vi "SelectByUID.vi"(8 "error in (no error)":errorcluster, 10 "UID":i32, 11 "appended array":refnum<vi>[](array[refnum])) -> (0 "error out":errorcluster, 3 "GObject out":refnum<vi>)   [LabVIEW 2020]
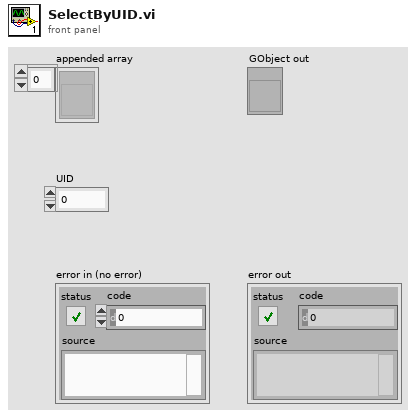
[diagram p1: front panel]
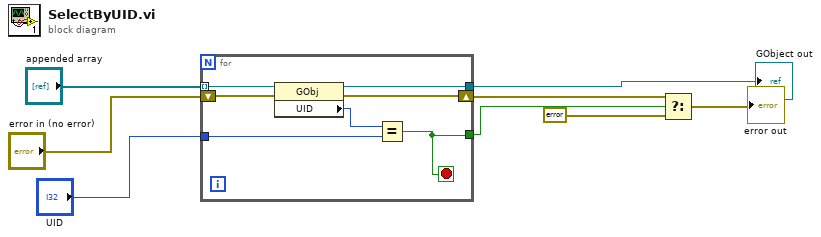
[diagram p0: block diagram]
diagram:
  n1 = for {
    tunnel: "appended array" -> [w15] mode=indexing
    tunnel: "UID" -> [w13]
    tunnel: [w12] -> w3
    tunnel: [w11] -> w7
    shift-right: [w9] -> w6
    shift-left: "error in (no error)" -> [w10]
    stop <- w11 stop-if-true
    n2 = property class="GObj"(reference=w15, error in=w10) -> (reference out=w12:refnum<vi>, error out=w9:errorcluster, "UID"=w14:i32)
    n3 = Equal?(x=w14, y=w13) -> (x = y?=w11:bool)
  }
  "GObject out" <- w3
  n4 = Select(t=w6, s=w7, f=errorcluster {"status"=TRUE, "code"=-1, "source"="GObject with ID not found"}) -> (s? t:f=→"error out":errorcluster)
